vi "Parse autobuild spec.vi"(8 "error in":errorcluster, 11 "Autobuild spec":path) -> (0 "error out":errorcluster, 3 "Tasks":T1[](array[typedef]), 5 "Retain Build":bool)   [LabVIEW 2010]
uses:
  Types/Job Type.ctl
  Types/Task Info.ctl
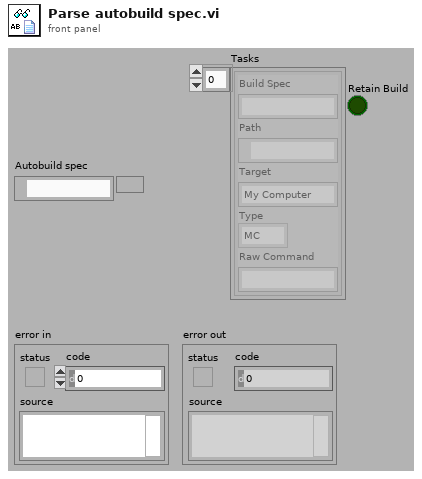
[diagram p1: front panel]
types:
  T1 = typedef "Task Info.ctl" = cluster{"Build Spec":string, "Path":path, "Target":string, "Type":T2, "Raw Command":string}
  T2 = typedef "Job Type.ctl" = enum16{"MC", "NOP", "VI", "Build", "VIP", "VIPB", "VIA"}
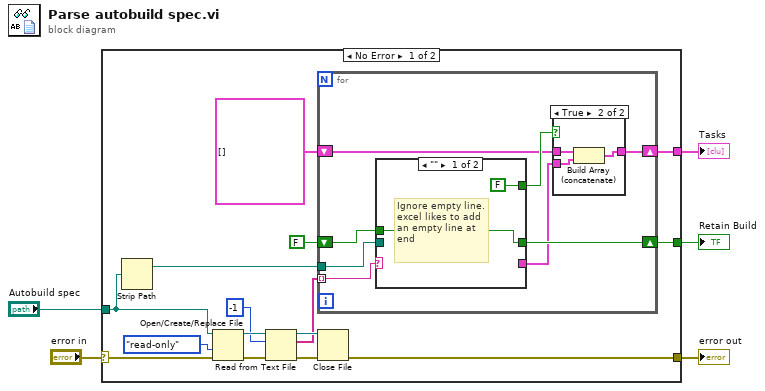
[diagram p0: block diagram]
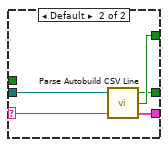
[diagram p3: hidden frame]
diagram:
  n1 = case shown="No Error" "error in" {
    selector: "error in" -> [w14 w40]
    tunnel: [w13 w40] -> w4
    tunnel: "Autobuild spec" -> [w11 _]
    tunnel: [w8 _] -> w2
    tunnel: [w7 _] -> w1
    frame No Error {
      n2 = Strip Path(path=w11) -> (stripped path=w10:path)  [unwired: 1 out]
      n3 = Open/Create/Replace File(file path (use dialog)=w11, error in=w14, access (0:read/write)=enum16{"read/write", "read-only", "write-only"}."read-only") -> (refnum out=w19:refnum<file>, error out=w18:errorcluster)  [unwired: 3 in, 1 out]
      n4 = Read from Text File(file (use dialog)=w19, count=-1, error in=w18) -> (refnum out=w16:refnum<file>, text=w12:string[], error out=w15:errorcluster)  [unwired: 1 in, 1 out]
      n5 = for {
        tunnel: w12 -> [w27] mode=indexing
        tunnel: w10 -> [w28]
        shift-right: [w25] -> w8
        shift-left: FALSE ("Retain Build") -> [w26]
        shift-right: [w22] -> w7
        shift-left: T1[] [] -> [w21]
        n6 = case shown="\"\"" w27 {
          selector: w27 -> [_ w37]
          tunnel: [_ w39] -> w23
          tunnel: w28 -> [_ w38]
          tunnel: [FALSE w36] -> w24
          tunnel: [w33 w35] -> w25
          tunnel: w26 -> [w33 _]
          frame "" {
            # "Ignore empty line. excel likes to add an empty line at end"
          }
          frame Default {
            n7 = call "Parse Autobuild CSV Line.vi"("String"=w37, "Autobuild root dir"=w38) -> ("Task Info"=w39:T1, "Build Command"=w36:bool, "Retain Build"=w35:bool)  [unwired: 1 in]
          }
        }
        n8 = case shown="True" w24 {
          tunnel: w23 -> [_ w31]
          tunnel: [w29 w32] -> w22
          tunnel: w21 -> [w29 w30]
          frame False {
          }
          frame True {
            n9 = Build Array (concatenate)(w30, w31) -> (w32:T1[])
          }
        }
      }
      n10 = Close File(refnum=w16, error in=w15) -> (error out=w13:errorcluster)  [unwired: 1 out]
    }
    frame Error {
    }
  }
  "error out" <- w4
  "Tasks" <- w1
  "Retain Build" <- w2
